vi "Test Double It.vi"() -> ()   [LabVIEW 2026]
doc: "Caraya unit test for Double It.vi\\2C generated by lvai_generate_test.\\0A\\0AOne static subVI call per case. Every assertion takes its error in from Define Test rather than from the assertion before it\\2C so a failing case cannot stop a later one - chaining them silently loses cases\\2C measured.\\0A\\0AThe error cluster carries the FIRST failure only. Read the JUnit report for all of them."
uses:
  <vilib>/addons/_JKI Toolkits/Caraya/classes/Test/Test.lvclass
  <vilib>/addons/_JKI Toolkits/Caraya/classes/Assert/Assert.lvclass
panel:
  out "error out":errorcluster
  in  "error in":errorcluster
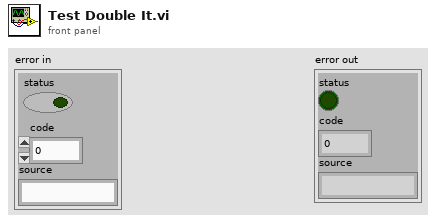
[diagram p1: front panel]
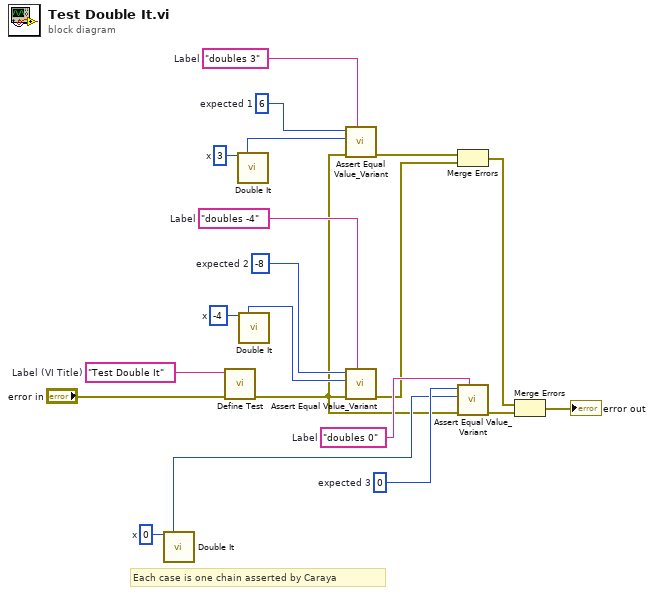
[diagram p0: block diagram]
diagram:
  w17 = "doubles 0"  # Label
  w16 = 0  # expected 3
  w14 = 0  # x
  w12 = "doubles -4"  # Label
  w11 = -8  # expected 2
  w9 = -4  # x
  w7 = "doubles 3"  # Label
  w6 = 6  # expected 1
  w4 = 3  # x
  w2 = "Test Double It"  # Label (VI Title)
  # "Each case is one chain asserted by Caraya"
  n1 = call "Double It.vi"("x"=w14) -> ("Doubled"=w15:i32)  [unwired: 14 in]
  n2 = call <vilib>:"Define Test.vi"("error in (no error)"="error in", "Label (VI Title)"=w2) -> ("error out"=w3:errorcluster)  [unwired: 8 in, 1 out]
  n3 = call "Double It.vi"("x"=w4) -> ("Doubled"=w5:i32)  [unwired: 14 in]
  n4 = call "Double It.vi"("x"=w9) -> ("Doubled"=w10:i32)  [unwired: 14 in]
  n5 = call <vilib>:"Assert Equal Value_Variant.vi"("Label"=w7, "error in (no error)"=w3, "Actual"=w5, "Expected"=w6) -> ("error out"=w8:errorcluster)  [unwired: 6 in, 1 out]
  n6 = call <vilib>:"Assert Equal Value_Variant.vi"("Label"=w12, "error in (no error)"=w3, "Actual"=w10, "Expected"=w11) -> ("error out"=w13:errorcluster)  [unwired: 6 in, 1 out]
  n7 = Merge Errors(w8, w13) -> (w19:errorcluster)
  n8 = call <vilib>:"Assert Equal Value_Variant.vi"("Label"=w17, "error in (no error)"=w3, "Actual"=w15, "Expected"=w16) -> ("error out"=w18:errorcluster)  [unwired: 6 in, 1 out]
  n9 = Merge Errors(w19, w18) -> (→"error out":errorcluster)
